vi "Set GPIO Number.vi"(8 "error in (no error)":errorcluster, 10 "GPIO Number":T1=-1, 11 "CTI_GPIO in":refnum<class "CTI_GPIO.lvclass">) -> (0 "error out":errorcluster, 3 "CTI_GPIO out":refnum<class "CTI_GPIO.lvclass">)   [LabVIEW 2021, in "CTI_GPIO.lvclass"]
uses:
  CTI_GPIO.lvclass
  <vilib>/CTI/CTI Drivers/CTI/GPIO Number.ctl
  <vilib>/CTI/CTI Drivers/CTI/CTI.lvlib
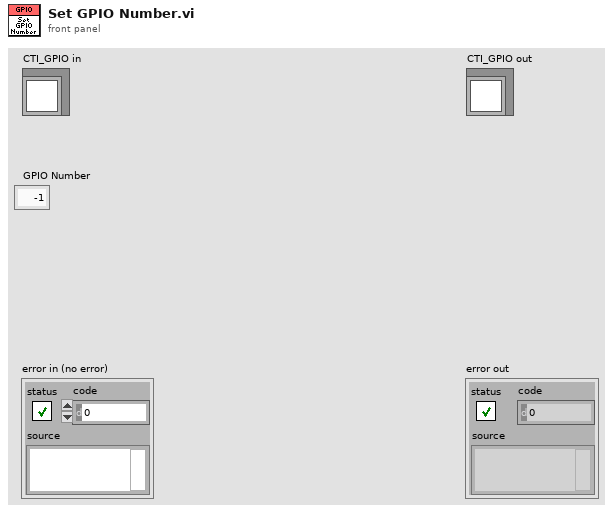
[diagram p1: front panel]
types:
  T1 = typedef "CTI.lvlib/GPIO Number.ctl" = i8
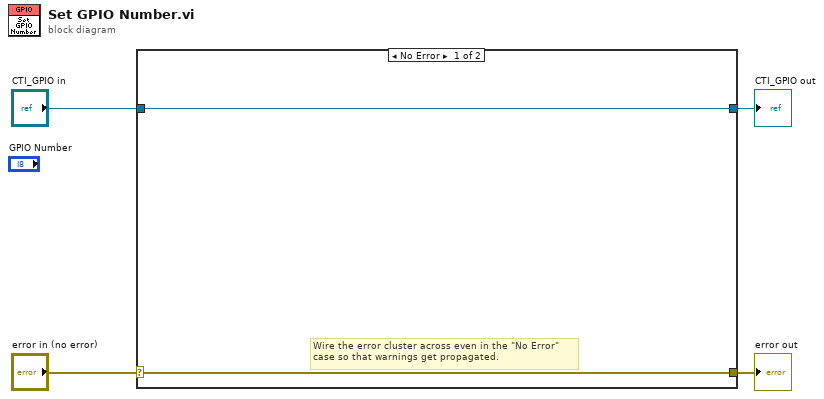
[diagram p0: block diagram]
diagram:
  n1 = case shown="No Error" "error in (no error)" {
    selector: "error in (no error)" -> [w5 w8]
    tunnel: [w5 w8] -> w3
    tunnel: [w6 w7] -> w1
    tunnel: "CTI_GPIO in" -> [w6 w7]
    frame No Error {
      # "Wire the error cluster across even in the \"No Error\"\ncase so that warnings get propagated."
    }
    frame Error {
    }
  }
  "error out" <- w3
  "CTI_GPIO out" <- w1
